vi "Update.vi"(8 "error in (no error)":errorcluster, 10 "Audio Data In":dbl[][](array[numeric]), 11 "Echo in":refnum<class "Echo.lvclass">) -> (0 "error out":errorcluster, 2 "Audio Data Out":dbl[][](array[numeric]), 3 "Echo out":refnum<class "Echo.lvclass">)   [LabVIEW 2019, in "Echo.lvlib" / "Echo.lvclass"]
doc: "Applies an echo effect to the audio. A delayed copy of the audio signal is added to the original signal. The resulting signal is output, but also stored in <b>Audio History Buffer Out</b> for reuse in subsequent iterations.\n\n<b>Value1:</b> Feedback amount\n<b>Value2:</b> Echo delay"
uses:
  Echo.lvclass
  Packed Libraries/Globals.lvlibp/Constants.vi
  Plugin Interfaces/Effect Interface/Effect Interface.lvlibp/Effect Interface Class/Effect Interface.lvclass
  Packed Libraries/Globals.lvlibp
  C:/github/dataflowg/dataflow-dj/src/Plugin Interfaces/Effect Interface/Effect Interface.lvlibp/Effect Interface Class/Effect Interface.lvclass
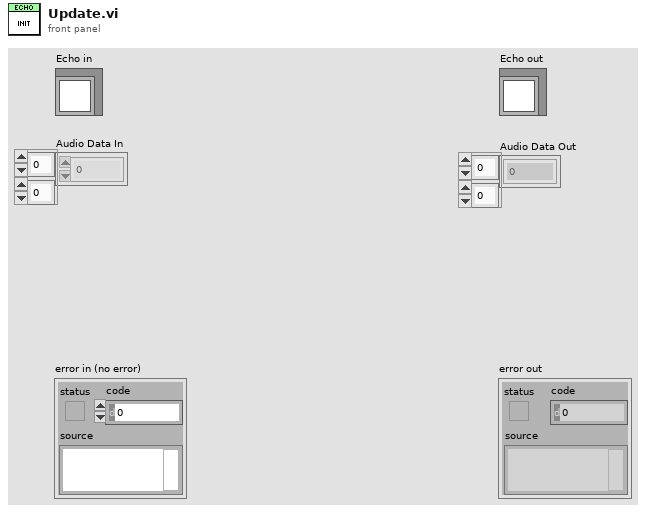
[diagram p1: front panel]
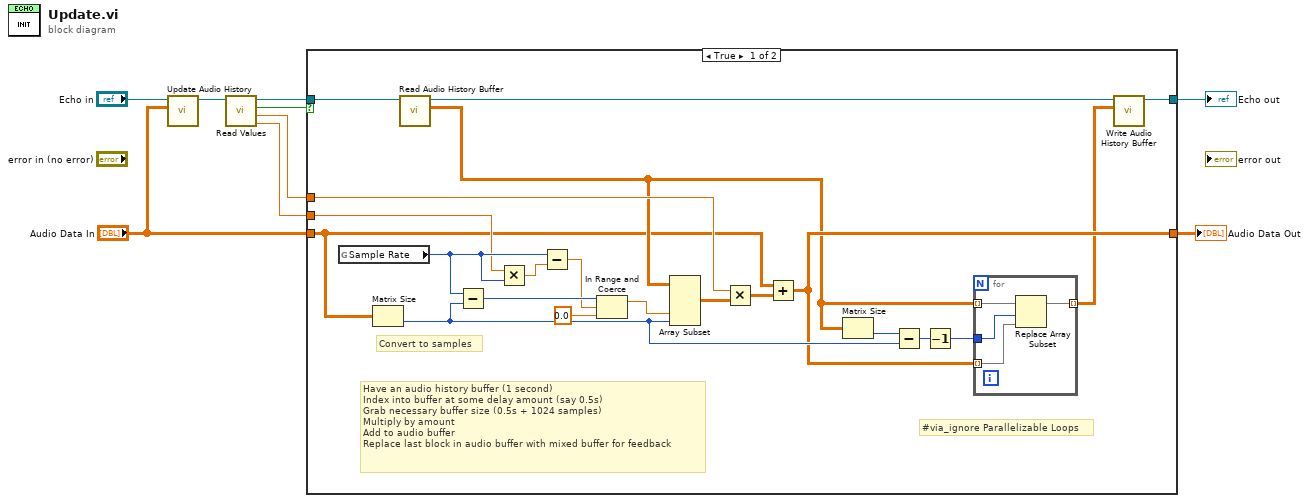
[diagram p0: block diagram]
diagram:
  n1 = call "Update Audio History.vi"("Audio Data In"="Audio Data In", "Effect Interface in"="Echo in") -> ("Effect Interface out"=w2:refnum<class "Echo.lvclass">)  [unwired: 8 in, 1 out]
  n2 = call "Read Values.vi"("Effect Interface in"=w2) -> ("Value2"=w4:dbl, "Value1"=w5:dbl, "Enable"=w6:bool, "Effect Interface out"=w8:refnum<class "Echo.lvclass">)  [unwired: 7 in]
  n3 = case shown="True" w6 {
    tunnel: [w18 w35] -> w9
    tunnel: w5 -> [w17 _]
    tunnel: w4 -> [w16 _]
    tunnel: "Audio Data In" -> [w11 w35]
    tunnel: w8 -> [w10 w36]
    tunnel: [w12 w36] -> w7
    frame True {
      # "#via_ignore Parallelizable Loops"
      # "Convert to samples"
      # "Have an audio history buffer (1 second)\nIndex into buffer at some delay amount (say 0.5s)\nGrab necessary buffer size (0.5s + 1024 samples)\nMultiply by amount\nAdd to audio buffer\nReplace last block in audio buffer with mixed buffer for feedback"
      n4 = global read "Constants.vi" "Sample Rate"() -> (w19:i32)
      n5 = Matrix Size(0:w11) -> (2:w24:i32)  [unwired: 1 out]
      n6 = call "Read Audio History Buffer.vi"("Effect Interface in"=w10) -> ("Audio History Buffer"=w15:dbl[][], "Effect Interface out"=w13:refnum<class "Echo.lvclass">)  [unwired: 9 in]
      n7 = Subtract(x=w19, y=w24) -> (x-y=w23:i32)
      n8 = Multiply(x=w16, y=w19) -> (x*y=w30:dbl)
      n9 = Subtract(x=w19, y=w30) -> (x-y=w22:dbl)
      n10 = In Range and Coerce(upper limit=w23, x=w22, lower limit=0.0) -> (coerced(x)=w20:dbl)  [unwired: 1 out]
      n11 = Array Subset(array=w15, index (col)=w20, length (col)=w24) -> (w29:dbl[][])  [unwired: 2 in]
      n12 = Multiply(x=w17, y=w29) -> (x*y=w28:dbl[][])
      n13 = Add(x=w11, y=w28) -> (x+y=w18:dbl[][])
      n14 = Matrix Size(0:w15) -> (2:w27:i32)  [unwired: 1 out]
      n15 = Subtract(x=w27, y=w24) -> (x-y=w26:i32)
      n16 = Decrement(x=w26) -> (x-1=w25:i32)
      n17 = for {
        tunnel: w25 -> [w33]
        tunnel: w15 -> [w34] mode=indexing
        tunnel: [w32] -> w14 mode=indexing
        tunnel: w18 -> [w31] mode=indexing
        n18 = Replace Array Subset(array=w34, new element=w31, index=w33) -> (w32:dbl[])
      }
      n19 = call "Write Audio History Buffer.vi"("Audio History Buffer"=w14, "Effect Interface in"=w13) -> ("Effect Interface out"=w12:refnum<class "Echo.lvclass">)  [unwired: 9 in]
    }
    frame False {
    }
  }
  "Audio Data Out" <- w9
  "Echo out" <- w7
